vi "MSG display box_Two_button_Configurable.vi"(4 "Button 2 Text":string="Cancel", 6 "Button 1 Text":string="OK", 8 "error in":errorcluster, 9 "Enable":bool=TRUE, 10 "input string":string) -> (0 "error out":errorcluster, 3 "Result":bool)   [LabVIEW 2021]
panel:
  in  "Button1":bool
  in  "Button 2":bool
  out "String":string
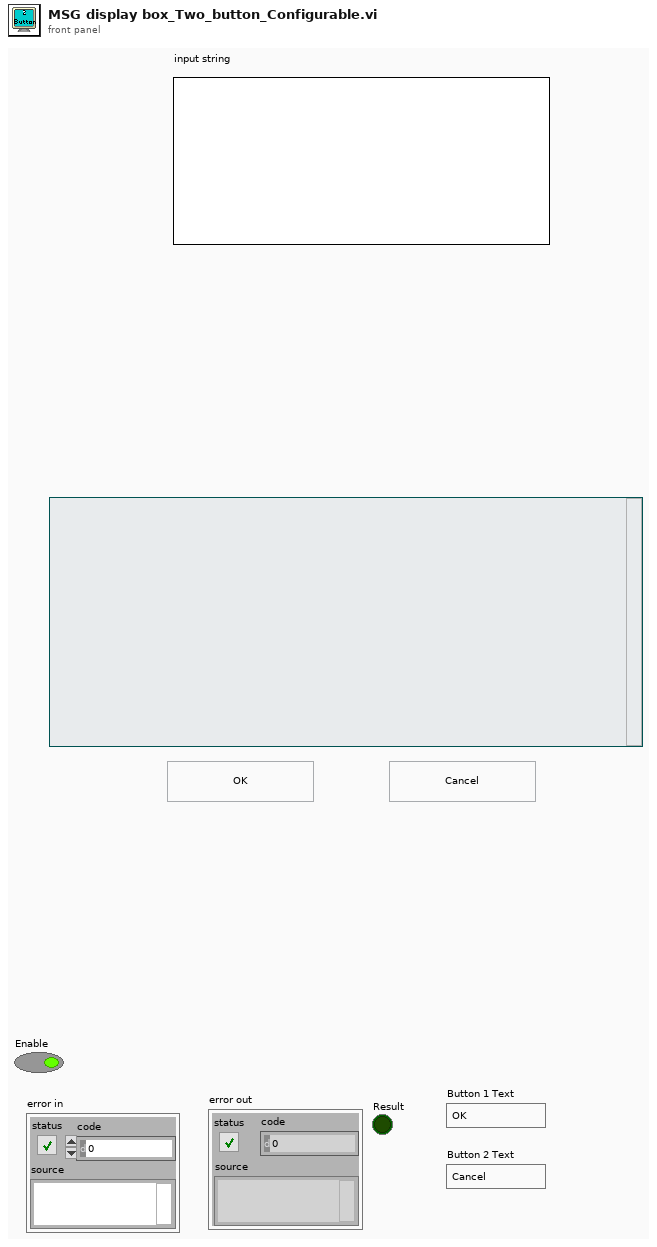
[diagram p1: front panel]
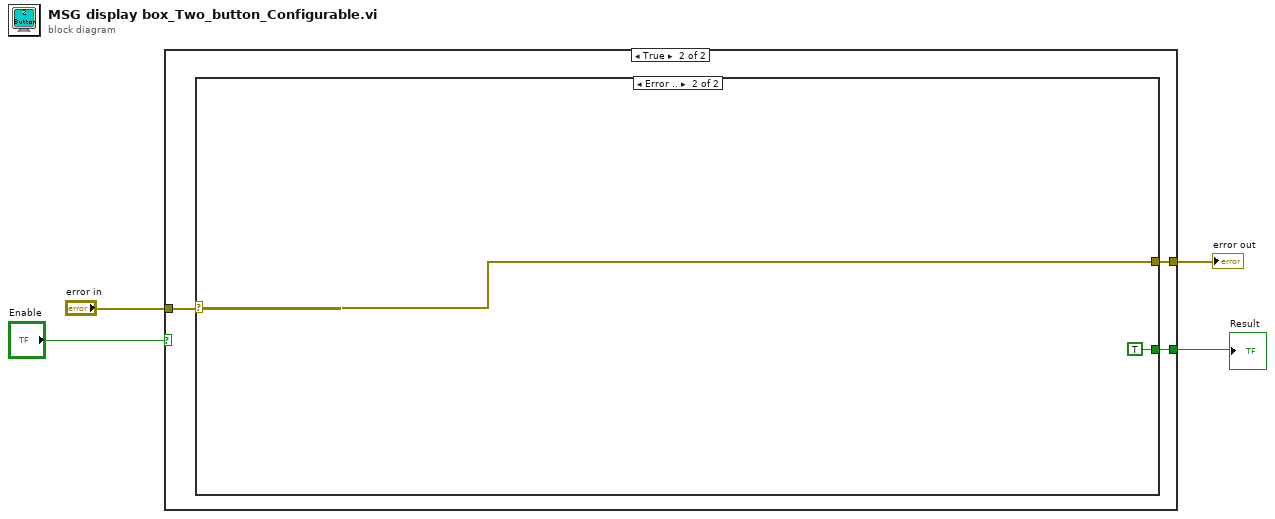
[diagram p0: block diagram]
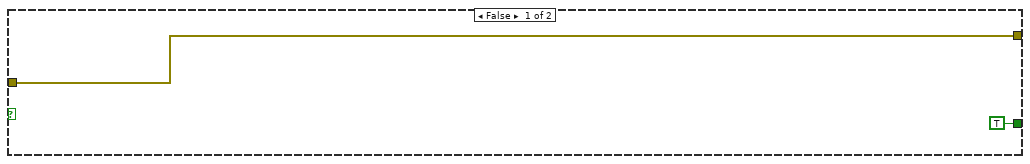
[diagram p2: hidden frame]
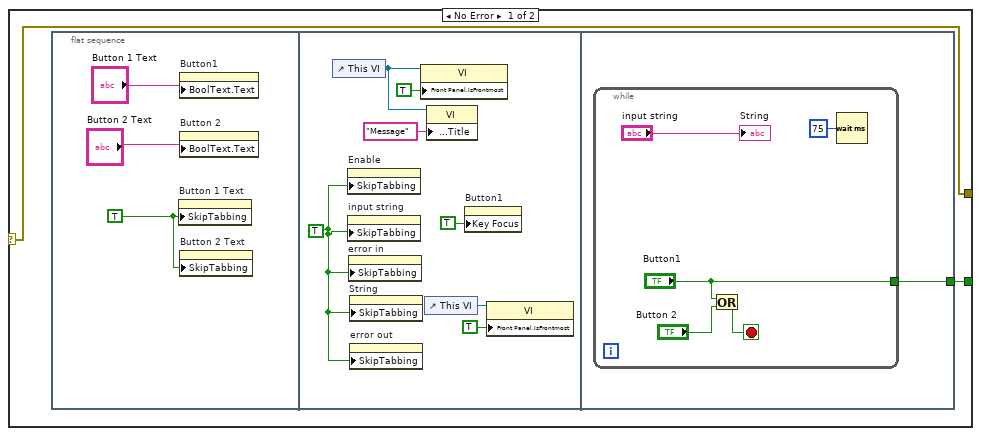
[diagram p3: hidden frame]
diagram:
  n1 = case shown="True" "Enable" {
    tunnel: "error in" -> [w6 w9]
    tunnel: [w6 w8] -> w3
    tunnel: [TRUE ("Button1") w7] -> w1
    frame False {
    }
    frame True {
      n2 = case shown="Error .." w9 {
        selector: w9 -> [w11 w29]
        tunnel: [w11 w29] -> w8
        tunnel: [w10 TRUE ("Button1")] -> w7
        frame No Error {
          n3 = flat-sequence {
            tunnel: [w22] -> w10
            frame #0 {
              w12 = TRUE ("Skip When Tabbing")
              n4 = property on="Button 1 Text" class="Str"("SkipTabbing"=w12) -> ()  [unwired: 2 in, 2 out]
              n5 = property on="Button1" class="Bool"("BoolText.Text"="Button 1 Text") -> ()  [unwired: 2 in, 2 out]
              n6 = property on="Button 2" class="Bool"("BoolText.Text"="Button 2 Text") -> ()  [unwired: 2 in, 2 out]
              n7 = property on="Button 2 Text" class="Str"("SkipTabbing"=w12) -> ()  [unwired: 2 in, 2 out]
            }
            frame #1 {
              w20 = TRUE ("Skip When Tabbing")
              n8 = control-ref of="This VI"() -> (w19:refnum<vi>)
              n9 = property on="Enable" class="Bool (strict)"("SkipTabbing"=w20) -> ()  [unwired: 2 in, 2 out]
              n10 = property on="input string" class="Str"("SkipTabbing"=w20) -> ()  [unwired: 2 in, 2 out]
              n11 = property on="error in" class="Clust (strict)"("SkipTabbing"=w20) -> ()  [unwired: 2 in, 2 out]
              n12 = property on="String" class="Str"("SkipTabbing"=w20) -> ()  [unwired: 2 in, 2 out]
              n13 = property on="error out" class="Clust (strict)"("SkipTabbing"=w20) -> ()  [unwired: 2 in, 2 out]
              n14 = property class="VI"(reference=w19, "Front Panel.IsFrontmost"=TRUE ("Front Panel Window:Is Frontmost")) -> ()  [unwired: 1 in, 2 out]
              n15 = control-ref of="This VI"() -> (w16:refnum<vi>)
              n16 = property class="VI"(reference=w19, "Front Panel.Title"="Message" ("VI Name")) -> ()  [unwired: 1 in, 2 out]
              n17 = property on="Button1" class="Bool"("Key Focus"=TRUE) -> ()  [unwired: 2 in, 2 out]
              n18 = property class="VI"(reference=w16, "Front Panel.IsFrontmost"=TRUE ("Front Panel Window:Is Frontmost")) -> ()  [unwired: 1 in, 2 out]
            }
            frame #2 {
              n19 = while {
                tunnel: ["Button1"] -> w22
                stop <- w25 stop-if-true
                n20 = Or(x="Button1", y="Button 2") -> (x .or. y?=w25:bool)
                n21 = Wait (ms)(milliseconds to wait=u32 75) -> ()  [unwired: 1 out]
                "String" <- "input string"
              }
            }
          }
        }
        frame Error {
        }
      }
    }
  }
  "error out" <- w3
  "Result" <- w1
